vi "FluidtekPrensaCONidentLEDI_v17.vi"() -> ()   [LabVIEW 2026]
uses:
  <vilib>/DAQmx/write.llb/DAQmx Write (Analog DBL 1Chan 1Samp).vi
  <vilib>/DAQmx/read.llb/DAQmx Read (Analog 2D DBL NChan NSamp).vi
  <vilib>/DAQmx/read.llb/DAQmx Read (Digital 1D Bool NChan 1Samp 1Line).vi
  <vilib>/DAQmx/write.llb/DAQmx Write (Digital 1D Bool NChan 1Samp 1Line).vi
  <extravilib>/ChannelInstances/Stream-a[15](dbl)/Read With Abort.vi
  <extravilib>/ChannelInstances/Tag-a[28](dbl)/Read With Abort.vi
  <extravilib>/ChannelInstances/Tag-a[.](dbl)/Write With Abort.vi
  <extravilib>/ChannelInstances/Tag-a[.](dbl)/Read With Abort.vi
  <extravilib>/ChannelInstances/Stream-a[15](dbl)/Write With Abort.vi
  <extravilib>/ChannelInstances/Tag-a[28](dbl)/Write With Abort.vi
  <extravilib>/ChannelInstances/Stream-a[15](dbl)/EndpointRead.vi
  <extravilib>/ChannelInstances/Stream-a[15](dbl)/Endpoint.vi
  GlobalesPrensa.vi
  <vilib>/Utility/file.llb/Write Delimited Spreadsheet (DBL).vi
  <vilib>/DAQmx/create/channels.llb/DAQmx Create Channel (AO-Voltage-Basic).vi
  <vilib>/DAQmx/miscellaneous.llb/DAQmx Fill In Error Info.vi
  <vilib>/DAQmx/create/channels.llb/DAQmx Create Channel (AI-Voltage-Basic).vi
  <vilib>/DAQmx/configure/timing.llb/DAQmx Timing (Sample Clock).vi
  <vilib>/DAQmx/create/channels.llb/DAQmx Create Channel (DO-Digital Output).vi
  <vilib>/DAQmx/create/channels.llb/DAQmx Create Channel (DI-Digital Input).vi
  <extravilib>/ChannelInstances/Tag-a[.](dbl)/Instantiate.vi
  <extravilib>/ChannelInstances/Stream-a[15](dbl)/Instantiate.vi
  <extravilib>/ChannelInstances/Stream-a[15](dbl)/)Channel.vi
  <resource>/ChannelSupport/_ChannelSupport/WaitIfNeeded.vi
  <extravilib>/ChannelInstances/Tag-a[28](dbl)/Instantiate.vi
  <extravilib>/ChannelInstances/Tag-a[28](dbl)/EndpointRead.vi
  <extravilib>/ChannelInstances/Tag-a[.](dbl)/Endpoint.vi
  <extravilib>/ChannelInstances/Tag-a[.](dbl)/EndpointRead.vi
  <extravilib>/ChannelInstances/Tag-a[28](dbl)/Endpoint.vi
  <extravilib>/ChannelInstances/Tag-a[28](dbl).lvlib
  <extravilib>/ChannelInstances/Tag-a[.](dbl).lvlib
  <extravilib>/ChannelInstances/Stream-a[15](dbl).lvlib
  <vilib>/ptbypt/NI_PtbyPt.lvlib
panel:
  out "Archivo":path
  in  "PARO DE EMERGENCIA":bool
  out "time/iteration (ms)":u32=210
  in  "Tab Control 3":enum32{"ENSAYO", "REGISTRO"}(tab)
  in  "Tipo ensayos":u16(ring)=1 items=["Flexotraccion en losas", "Tenacidad Vigas"]
  in  "Rampa (mm/min)":dbl=0.1 min=0.0 max=30.0 format="%.3f"
  in  "Rampa (kN/min)":dbl=0.1 min=0.0 max=20.0 format="%.2f"
  in  "Limite fuerza (kN)":dbl=3.0 min=0.0 max=150.0 format="%.2f"
  in  "Limite posicion (mm)":dbl=145.0 min=0.0 max=150.0 format="%.2f"
  in  "Tiempo carga (s)":dbl=3.0 min=0.0 max=300.0 format="%.2g"
  out "Tiempo (s)":dbl format="%.2f"
  in  "Iniciar ensayo":bool
  out "Velocidad norma (mm/min)  2":string="0.05 - 0.1"
  in  "Tenacidad en vigas":u16(ring) items=["ASTM 1609 con100x100x350", "ASTM 1609 con150x150x500", "EFNARC 1996", "VIGAS 14651", "ENS. BARCELONA"]
  in  "Aplicar velocidad de norma":bool
  out "Estado del ensayo":dbl(ring) items=["REPOSO", "CARGA (rampa)", "MANTENIENDO CARGA", "DESCARGA", "RETORNO / FIN", "FALLA - ENSAYO DETENIDO", ""]
  in  "Flexotracción en losas":u16(ring)=3 items=["EFNARC 1996", "EFNARC 1999", "EFNARC 14488-5", "ASTM 1550"]
  out "Velocidad norma (mm/min)":dbl=4.0
  in  "IPAddress QuantumX":string="172.31.236.115"
  out "LicenseIsValid":bool
  in  "Registrar":bool
  in  "ID manual (0=auto)":i32
  in  "Tipo":string
  in  "INFLE":dbl
  in  "Detener registro":bool
  in  "Tab Control 2":T1(tab)
  out "Presión B (bar)":dbl=31.47939829954219 format="%.2f"
  out "Presión A (bar)":dbl=47.7049180327869 format="%.2f"
  out "Vertical Progress Bar":dbl(slide)=3.0
  in  "Tab Control":enum32{"Desplazamiento", "Fuerza"}(tab)
  out "control signals":dynamicdata(graph)=[{"t0"=timestamp(3594752785.1434503 s since 1904-01-01), "dt"=1.0, "Y"=[3.0]}, {"t0"=timestamp(3594752785.1434503 s since 1904-01-01), "dt"=1.0, "Y"=[3.0680651042487943]}]
  in  "Posicion deseada (mm)":dbl(slide)=3.0 min=2.0 max=150.0 scale format="%#_2f"
  in  "Fuerza deseada (kN)":dbl=0.5 min=0.0 max=150.0 format="%.2f"
  out "Fuerza actual (KN)":dbl format="%.2f"
  out "Posicion actual (mm)":dbl format="%.2f"
  in  "Tipo control":u16(ring) items=["Desplazamiento", "Fuerza"]
  out "fuerza desplazamiento":cluster{dbl[], dbl[]}(graph)
  out "Rigidez estimada (kN/mm)":dbl
  out "Carga maxima (kN)":dbl
  out "Progreso mantenimiento":dbl(slide) scale=0.0..100.0
  out "Tiempo restante carga (s)":dbl
  out "Falla":bool
  out "Causa de la falla":dbl(ring) items=["Sin falla", "CAIDA DE CARGA (rotura)", "SOBRECARGA", "LIMITE DE POSICION", "PARO DE EMERGENCIA", "LIMITE DEL SISTEMA (160 kN)", "BOMBA DETENIDA", "LIMITE POR PRESIONES (160 kN)"]
  out "Proteccion de fuerza activa":bool
  in  "Vel. aproximacion (mm/min)":dbl=50.0 min=0.1 max=50.0
  in  "Fmax fuera de ensayo (kN)":dbl=1.0 min=0.2 max=50.0
  out "UPH energizada":bool=TRUE
  out "Nivel tanque":bool
  out "Estado de  filtro":bool=TRUE
  out "Sobrecorriente":bool
  in  "Stop":bool
  out "Estado de motor":bool
  in  "Apagar":bool
  in  "Encender":bool
  in  "Sin proteccion de carga":bool
  out "Consigna posicion interna (mm)":dbl
  out "Parametros avanzados":dbl(ring) items=["POR DEFECTO (bloqueados)", "PERSONALIZADOS (activos)"]
  in  "Codigo acceso":dbl
  in  "Kf lazo fuerza (1/s)":dbl=0.5
  in  "Kx lazo posicion (V/mm)":dbl=30.0
  in  "Ti lazo posicion (s)":dbl=1.5
  # "PB"
  # "PA"
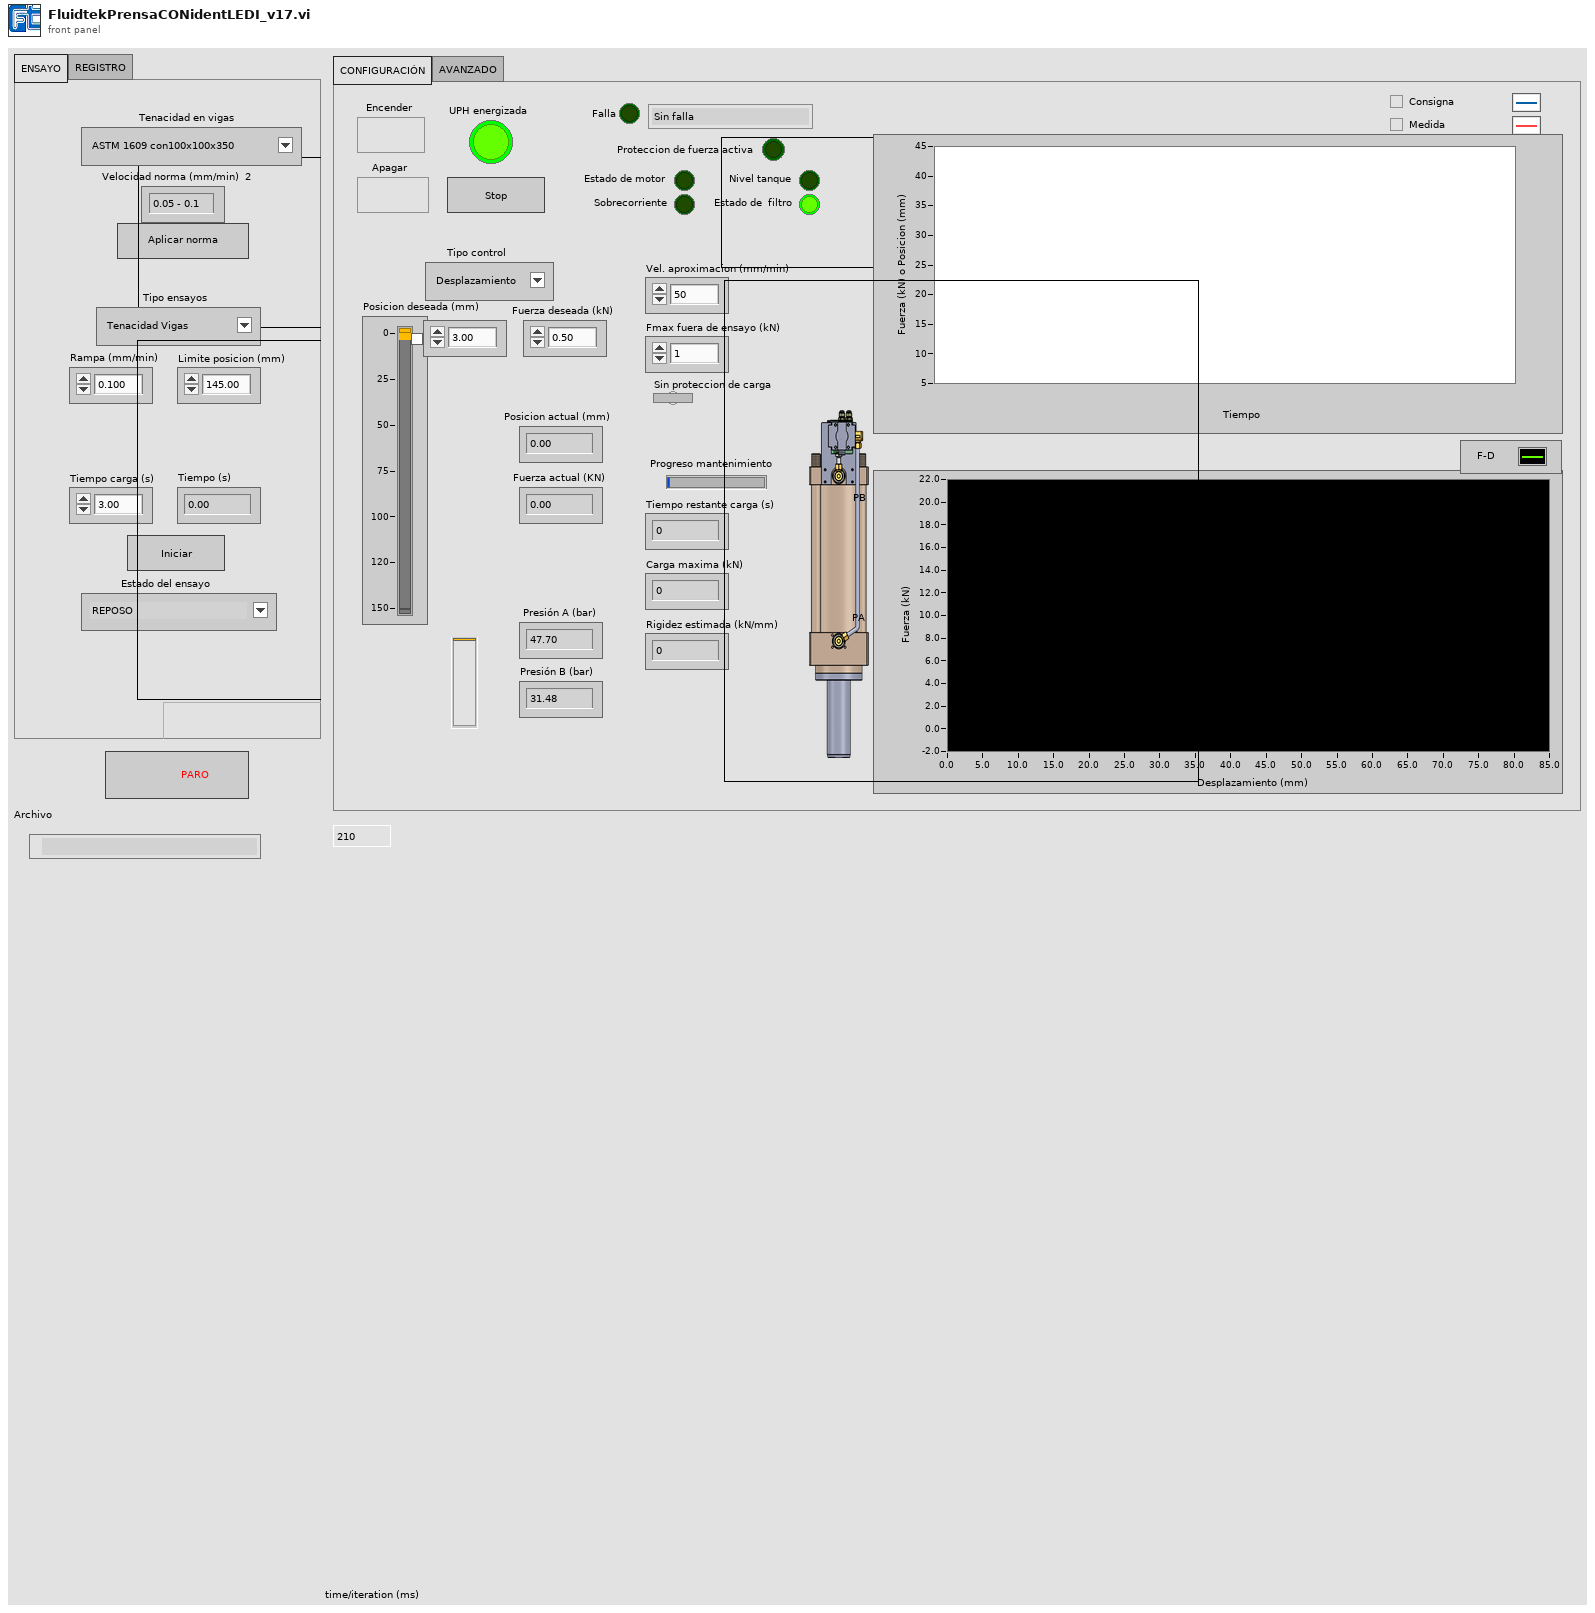
[diagram p1: front panel]
types:
  T1 = enum32{"CONFIGURACIÓN", "AVANZADO", "identificación (no modificar)"}
  T2 = cluster{"Devices":refnum<k24>[], "Signals":refnum<k24>[]}
  T3 = typedef "Tag-a[28](dbl).lvlib/))Channel.ctl" = refnum<queue>
  T4 = typedef "Stream-a[15](dbl).lvlib/)Channel.ctl" = refnum<queue>
  T5 = enum8{"Enabled", "Disabled", "Disabled and Grayed Out"}
  T6 = typedef "Tag-a[.](dbl).lvlib/))Channel.ctl" = refnum<queue>
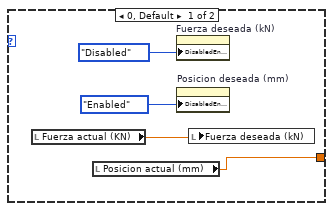
[diagram p9: hidden frame]
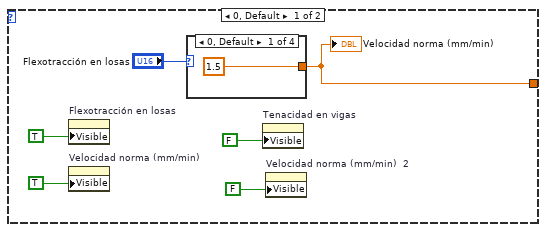
[diagram p10: hidden frame]
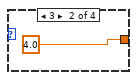
[diagram p11: hidden frame]
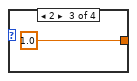
[diagram p12: hidden frame]
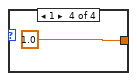
[diagram p13: hidden frame]
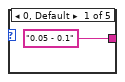
[diagram p14: hidden frame]
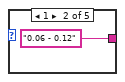
[diagram p15: hidden frame]
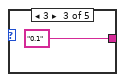
[diagram p16: hidden frame]
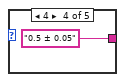
[diagram p17: hidden frame]
diagram:
  w93 = 0 items=["one channel for each line", "one channel for all lines"] ("line grouping")
  w100 = 0 items=["one channel for each line", "one channel for all lines"] ("line grouping")
  w103 = 10348 items=["Volts"=10348, "From Custom Scale"=10065] ("units")
  w106 = -1 items=["Default"=-1, "RSE"=10083, "NRSE"=10078, "Differential"=10106, "Pseudodifferential"=12529] ("input terminal configuration")
  w114 = 10348 items=["Volts"=10348, "From Custom Scale"=10065] ("units")
  w112 = 10106 items=["Default"=-1, "RSE"=10083, "NRSE"=10078, "Differential"=10106, "Pseudodifferential"=12529] ("input terminal configuration")
  w108 = 10123 items=["Finite Samples"=10178, "Continuous Samples"=10123, "Hardware Timed Single Point"=12522] ("sample mode")
  # "Convert device reference to array of device references\n(since ConnectDevice.vi expects an array of devices)..."
  # "Disconnect devices"
  # "Set samplerate and filter frequency for all selected signals."
  # "Initialize HBM Common API for LabVIEW"
  # "End API usage"
  # "Stop DAQ"
  # "Run data acquisition for 10 sec. DAQ-loop: Update signals and do anything with the  measurement values.\n(Here: show first signal in diagram)"
  # "Start DAQ"
  # "Prepare DAQ"
  # "v14: senales [0,1,2,3] -> lazo lee 1,2,3 = W100 (conector 2), Tempsonic (conector 3), Celda via Krenel (conector 4). Filtro 20 Hz, 50 Hz"
  # "Get all signals of the devices"
  # "Connect devices"
  # "Use certain QuantumX device"
  # "Assign the signals...."
  n1 = call <userlib>:"Init.vi"() -> ("LicenseIsValid"=→"LicenseIsValid":bool, "Error out"=w53:errorcluster)  [unwired: 8 in, 1 out]
  n2 = call <userlib>:"QuantumX_Device.vi"("Error in"=w53, "IPAddress"="IPAddress QuantumX") -> ("Error out"=w54:errorcluster, "Device"=w51:refnum<k24>)  [unwired: 6 in]
  n3 = Build Array(w51) -> (w50:refnum<k24>[])
  n4 = call <userlib>:"ConnectDevice.vi"("Error in"=w54, "Devices"=w50) -> ("Error out"=w76:errorcluster, "Devices"=w75:refnum<k24>[])  [unwired: 7 in, 1 out]
  n5 = call <userlib>:"GetSignals.vi"("Error in"=w76, "Devices"=w75) -> ("Error out"=w70:errorcluster, "DevicesAndSignals"=w71:T2)  [unwired: 8 in]
  n6 = Unbundle By Name(w71) -> ("Devices"=w64:refnum<k24>[], "Signals"=w68:refnum<k24>[])
  n7 = Index Array(array=w68, index #1=0 ("Index"), index #2=1 ("Index"), index #3=2 ("Index"), index #4=3 ("Index")) -> (element #1=w67:refnum<k24>, element #2=w66:refnum<k24>, element #3=w59:refnum<k24>, element #4=w58:refnum<k24>)
  n8 = Build Array(w67, w66, w59, w58) -> (w65:refnum<k24>[])
  n9 = Bundle(cluster=w71, "Devices"=w64, "Signals"=w65) -> (w72:T2)
  n10 = Unbundle By Name(w72) -> ("Signals"=w88:refnum<k24>[])
  n11 = case shown="No Error" w70 {
    tunnel: w70 -> [w122 w128]
    tunnel: w88 -> [w121 _]
    tunnel: [w120 w128] -> w87
    frame No Error {
      # "Filter frequency:"
      # "Samplerate:"
      n12 = for {
        tunnel: w122 -> [w127]
        tunnel: 50.0 ("SampleRate") -> [w126]
        tunnel: 20.0 ("FilterFrequency") -> [w125]
        tunnel: w121 -> [w124] mode=indexing
        tunnel: [w123] -> w120
        stop <- w123 stop-if-true
        n13 = call <userlib>:"ConfigSignal.vi"("Error in"=w127, "SampleRate"=w126, "FilterFrequency"=w125, "Signal"=w124) -> ("Error out"=w123:errorcluster)  [unwired: 7 in]
      }
    }
    frame Error {
    }
  }
  n14 = call <userlib>:"AssignSignals.vi"("Error in"=w87, "DevicesAndSignals"=w72) -> ("Error out"=w85:errorcluster, "DevicesAndSignals"=w86:T2)  [unwired: 8 in]
  n15 = call <userlib>:"PrepareDAQ.vi"("Error in"=w85, "DevicesAndSignals"=w86) -> ("Error out"=w82:errorcluster, "DaqMeasurement"=w83:refnum<k24>, "DevicesAndSignals"=w84:T2)  [unwired: 7 in]
  n16 = call <userlib>:"StartDaq.vi"("DevicesAndSignals"=w84, "DaqMeasurement"=w83, "AcquisitionMode"=2, "Error in"=w82) -> ("DevicesAndSignals"=w79:T2, "DaqMeasurement"=w80:refnum<k24>, "Error out"=w81:errorcluster)  [unwired: 7 in, 2 out]
  n17 = while {
    tunnel: w80 -> [w184]
    tunnel: w79 -> [w183]
    tunnel: [w179] -> w78
    tunnel: [w178] -> w77
    tunnel: w81 -> [w185]
    tunnel: [w177] -> w46
    shift-right: [w145] -> _
    shift-left: 0 -> [w170]
    shift-right: [w136] -> _
    shift-left: FALSE ("Registrar") -> [w141]
    shift-right: [w140] -> _
    shift-left: _ -> [w142]
    stop <- w131 stop-if-true
    n18 = global read "GlobalesPrensa.vi" "Salir"() -> (w130:bool)
    n19 = Get Date/Time In Seconds() -> (seconds since 1Jan1904=w153:timestamp)
    n20 = Format Into String(format string="D:\\\\%<%Y>T\\\\%03d-%<%Y>T", w153, "INFLE", w153) -> (resulting string=w155:string)  [unwired: 2 in, 1 out]
    n21 = Or(x=w130, y="Detener registro") -> (x .or. y?=w131:bool)
    n22 = String To Path(string=w155) -> (path=w158:path)
    n23 = Create Folder(path (use dialog)=w158) -> (error out=w156:errorcluster)  [unwired: 2 in, 2 out]
    n24 = Format Into String(format string="%s P*", "Tipo") -> (resulting string=w159:string)  [unwired: 2 in, 1 out]
    n25 = call <vilib>:"Clear Errors.vi"("error in (no error)"=w156) -> ("error out"=w157:errorcluster)  [unwired: 5 in, 1 out]
    n26 = List Folder(path=w158, pattern=w159, error in=w157) -> (path out=w168:path, filenames=w160:string[])  [unwired: 1 in, 2 out]
    n27 = Not(x=w141) -> (.not. x?=w147:bool)
    n28 = for {
      tunnel: w160 -> [w212] mode=indexing
      tunnel: [w210] -> w161 mode=indexing
      n29 = Scan From String(format string="%s P%d", input string=w212) -> (error out=w209:errorcluster, output 2=w210:i32)  [unwired: 5 in, 2 out]
      n30 = call <vilib>:"Clear Errors.vi"("error in (no error)"=w209) -> ()  [unwired: 5 in, 2 out]
    }
    n31 = Array Max & Min(array=w161) -> (max value=w162:i32)  [unwired: 3 out]
    n32 = Greater Than 0?(x="ID manual (0=auto)") -> (x > 0?=w164:bool)
    n33 = Increment(x=w162) -> (x+1=w163:i32)
    n34 = Select(t="ID manual (0=auto)", s=w164, f=w163) -> (s? t:f=w166:i32)
    n35 = global read "GlobalesPrensa.vi" "Ensayando"() -> (w137:bool)
    n36 = global read "GlobalesPrensa.vi" "InfoEnsayo"() -> (w134:string)
    n37 = Format Into String(format string="%s P%d.csv", "Tipo", w166) -> (resulting string=w167:string)  [unwired: 2 in, 1 out]
    n38 = Or(x="Registrar", y=w137) -> (x .or. y?=w136:bool)
    n39 = Build Path(base path=w168, name or relative path=w167) -> (appended path=w143:path)
    n40 = Get Date/Time In Seconds() -> (seconds since 1Jan1904=w135:timestamp)
    n41 = And(x=w136, y=w147) -> (x .and. y?=w148:bool)
    n42 = Select(t=w142, s=w141, f=w143) -> (s? t:f=w140:path)
    "Archivo" <- w140
    n43 = Format Into String(format string="Fecha\t%<%Y-%m-%d %H:%M:%S>T\nNorma\t%s\nFrecuencia (Hz)\t50\nRunning Time\tDeflection\tDisplacement\tLoad\ns\tmm\tmm\tkN\n", w135, w134) -> (resulting string=w133:string)  [unwired: 2 in, 1 out]
    n44 = case shown="True" w148 {
      tunnel: [_ w207] -> w149
      tunnel: w140 -> [_ w205]
      tunnel: w133 -> [_ w206]
      frame False {
      }
      frame True {
        (unwired) "" ("text")
        (unwired) errorcluster {"status"=FALSE, "code"=0, "source"=""} ("error in")
        (unwired) "" ("prompt (Choose or enter file path)")
        # "t (s)\\testado\\tconsigna\\tF (kN)\\tx (mm)\\txsp (mm)\\tu (V)\\tkh (kN/mm)\\tdt (s)\\tfalla\\tcausa\\tprot\\n"
        n45 = Path To String(path=w205) -> (string=w204:string)
        n46 = Search and Replace String(replace all?=FALSE ("replace all? (F)"), case sensitive?=FALSE ("ignore case? (F)"), input string=w204, search string=".csv", replace string="_control.csv" ("replace string (\"\")"), offset=0 ("offset (0)"), error in=errorcluster {"status"=FALSE, "code"=0, "source"=""} ("error in (no error)")) -> (result string=w197:string)  [unwired: 1 in, 3 out]
        n47 = String To Path(string=w197) -> (path=w196:path)
        n48 = Write to Text File(file (use dialog)=w196, text="t (s)\testado\tconsigna\tF (kN)\tx (mm)\txsp (mm)\tu (V)\tkh (kN/mm)\tdt (s)\tfalla\tcausa\tprot\tpA (bar)\tpB (bar)\tFp (kN)\n") -> (error out=w194:errorcluster)  [unwired: 2 in, 2 out]
        n49 = flat-sequence {
          tunnel: w196 -> [w208]
          tunnel: w194 -> [_]
          frame #0 {
            n50 = global write "GlobalesPrensa.vi" "ArchivoControl"(w208) -> ()
          }
        }
        n51 = Write to Text File(file (use dialog)=w205, text=w206) -> (error out=w207:errorcluster)  [unwired: 2 in, 2 out]
      }
    }
    n52 = call <userlib>:"UpdateMeasurementValues.vi"("Error in"=w185, "DaqMeasurement"=w184, "DevicesAndSignals"=w183) -> ("Error out"=w180:errorcluster, "DaqMeasurement"=w181:refnum<k24>, "DevicesAndSignals"=w182:T2)  [unwired: 6 in]
    n53 = for {
      N: 3 -> [_]
      shift-right: [w224] -> w178
      shift-left: w182 -> [w228]
      shift-right: [w225] -> w179
      shift-left: w181 -> [w227]
      shift-right: [w223] -> w177
      shift-left: w180 -> [w226]
      tunnel: [w218] -> w129 mode=indexing
      i -> [w221]
      n54 = Add(x=w221, y=1.0) -> (x+y=w220:dbl)
      n55 = call <userlib>:"GetMeasurementValues.vi"("Error in"=w226, "Index"=w220, "DaqMeasurement"=w227, "DevicesAndSignals"=w228) -> ("Error out"=w223:errorcluster, "Waveform"=w219:waveform(dbl), "DaqMeasurement"=w225:refnum<k24>, "DevicesAndSignals"=w224:T2)  [unwired: 2 in, 2 out]
      n56 = Unbundle By Name(w219) -> ("Y"=w218:dbl[])
    }
    n57 = Array Size(array=w129) -> (size(s)=w173:i32[])
    n58 = Index Array(array=w173, index=1) -> (element=w171:i32)
    n59 = for {
      N: w171 -> [_]
      tunnel: [w215] -> w169 mode=indexing
      tunnel: w170 -> [w213]
      i -> [w217]
      n60 = Add(x=w217, y=w213) -> (x+y=w216:i32)
      n61 = Multiply(x=w216, y=0.02) -> (x*y=w215:dbl)
    }
    n62 = Add(x=w170, y=w171) -> (x+y=w146:i32)
    n63 = Select(t=w146, s=w136, f=0) -> (s? t:f=w145:i32)
    n64 = case shown="True" w136 {
      tunnel: w129 -> [_ w193]
      tunnel: w169 -> [_ w192]
      tunnel: w149 -> [_ w187]
      tunnel: w140 -> [_ w186]
      frame False {
      }
      frame True {
        n65 = Insert Into Array(array=w193, index (row)=0, new element=w192) -> (w190:dbl[][])  [unwired: 1 in]
        n66 = call-poly <vilib>:"Write Delimited Spreadsheet.vi"("file path (dialog if empty)"=w186, "2D data"=w190, "append to file? (new file:F)"=TRUE, "error in (no error)"=w187, "transpose? (no:F)"=TRUE) -> ()  [unwired: 9 in, 2 out]
      }
    }
    n67 = Wait Until Next ms Multiple(millisecond multiple=u32 20 ("Vielfache von ms")) -> ()  [unwired: 1 out]
  }
  n68 = while {
    tunnel: [w230] -> w44
    tunnel: [w230] -> w43
    tunnel: [w230] -> w42
    i -> [w235]
    stop <- w233 continue-if-true
    n69 = call <vilib>:"DAQmx Reserve Network Device.vi"("device in"=tag "cDAQ9184-1ADC24C", "override reservation?"=TRUE, "error in"=errorcluster {"status"=FALSE, "code"=0, "source"=""}) -> ("error out"=w230:errorcluster)  [unwired: 11 in, 1 out]
    n70 = Unbundle By Name(w230) -> ("status"=w232:bool)
    n71 = Less?(x=w235, y=30) -> (x < y?=w234:bool)
    n72 = Wait (ms)(milliseconds to wait=u32 2000) -> ()  [unwired: 1 out]
    n73 = And(x=w232, y=w234) -> (x .and. y?=w233:bool)
  }
  n74 = call-poly <vilib>:"DAQmx Create Virtual Channel.vi"("maximum value"=10.0, "minimum value"=0.0, "input terminal configuration"=w112, "physical channels"=tag "PrensaLEDI_AI/ai0:3", "units"=w114, "error in"=w42) -> ("task out"=w115:refnum<k21>, "error out"=w116:errorcluster)  [unwired: 8 in]
  n75 = call-poly <vilib>:"DAQmx Create Virtual Channel.vi"("maximum value"=10.0, "minimum value"=-10.0, "output terminal configuration"=w106, "physical channels"=tag "PrensaLEDI_AO/ao0", "units"=w103, "error in"=w42) -> ("task out"=w107:refnum<k21>, "error out"=w105:errorcluster)  [unwired: 8 in]
  n76 = call-poly <vilib>:"DAQmx Create Virtual Channel.vi"("lines"=tag "PrensaLEDI_DI/port0/line0:7", "line grouping"=w100, "error in"=w44) -> ("task out"=w97:refnum<k21>, "error out"=w98:errorcluster)  [unwired: 11 in]
  n77 = call-poly <vilib>:"DAQmx Create Virtual Channel.vi"("lines"=tag "PrensaLEDI_DO/port0/line0:7", "line grouping"=w93, "error in"=w43) -> ("task out"=w94:refnum<k21>, "error out"=w95:errorcluster)  [unwired: 11 in]
  n78 = call <vilib>:"DAQmx Start Task.vi"("task/channels in"=w107, "error in"=w105) -> ("task out"=w40:refnum<k21>, "error out"=w41:errorcluster)  [unwired: 12 in]
  n79 = call <vilib>:"Clear Errors.vi"("error in (no error)"=w46) -> ("error out"=w45:errorcluster)  [unwired: 5 in, 1 out]
  n80 = call <vilib>:"DAQmx Start Task.vi"("task/channels in"=w97, "error in"=w98) -> ("task out"=w25:refnum<k21>, "error out"=w17:errorcluster)  [unwired: 12 in]
  n81 = call <vilib>:"DAQmx Start Task.vi"("task/channels in"=w94, "error in"=w95) -> ("task out"=w37:refnum<k21>, "error out"=w18:errorcluster)  [unwired: 12 in]
  n82 = call-poly <vilib>:"DAQmx Timing.vi"("task/channels in"=w115, "sample mode"=w108, "samples per channel"=500000, "rate"=200000.0, "error in"=w116) -> ("task out"=w92:refnum<k21>, "error out"=w91:errorcluster)  [unwired: 9 in]
  n83 = call <userlib>:"StopDaq.vi"("Error in"=w45, "DaqMeasurement"=w78, "DevicesAndSignals"=w77) -> ("Error out"=w57:errorcluster, "DevicesAndSignals"=w56:T2)  [unwired: 7 in]
  n84 = call-poly <vilib>:"DAQmx Write.vi"("task/channels in"=w40, "data"=-0.5, "error in"=w41) -> ("task out"=w36:refnum<k21>, "error out"=w15:errorcluster)  [unwired: 10 in, 1 out]
  n85 = call <vilib>:"DAQmx Start Task.vi"("task/channels in"=w92, "error in"=w91) -> ("task out"=w38:refnum<k21>, "error out"=w16:errorcluster)  [unwired: 12 in]
  n86 = call <userlib>:"DisconnectDevice.vi"("Error in"=w57, "DevicesAndSignals"=w56) -> ("Error out"=w55:errorcluster)  [unwired: 9 in]
  n87 = call <vilib>:"Simple Error Handler.vi"("error in (no error)"=w55) -> ("error out"=w74:errorcluster)  [unwired: 4 in, 4 out]
  n88 = Merge Errors(w18, w17, w16, w15) -> (w19:errorcluster)
  n89 = call <userlib>:"DisposeApi.vi"("Error in"=w74) -> ()  [unwired: 10 in, 1 out]
  n90 = global write "GlobalesPrensa.vi" "Salir"(FALSE ("Salir")) -> ()
  n91 = while {
    tunnel: w38 -> [w280]
    tunnel: w37 -> [w270]
    tunnel: w36 -> [w268]
    tunnel: dbl[] [0.0, 0.0, 0.0, 0.0, 0.0, 0.0, 0.0, 0.0, 0.0, 0.0, 0.0, 0.0, 0.0, 0.0, 0.0, 0.0, 0.0] -> [w265]
    tunnel: dbl[] [0.0, 0.0, 0.0, 0.0, 0.0, 0.0, 0.0, 0.0] -> [w264]
    tunnel: [w263] -> w32
    tunnel: [w262] -> w31
    tunnel: w25 -> [w260]
    tunnel: [w259] -> w22
    tunnel: [w258] -> w21
    tunnel: [w257] -> w20
    tunnel: w19 -> [w256]
    tunnel: [w243] -> w13
    tunnel: [w242] -> w2
    tunnel: w1 -> [w241]
    stop <- w244 stop-if-true
    n92 = call <extravilib>:"Read.vi"("channel"=w241) -> ("element"=w240:dbl[])  [unwired: 1 in, 1 out]
    n93 = call-poly <vilib>:"DAQmx Read.vi"("task/channels in"=w280, "number of samples per channel"=4000, "error in"=w256) -> ("task out"=w258:refnum<k21>, "data"=w279:dbl[][], "error out"=w255:errorcluster)  [unwired: 10 in]
    n94 = call-poly <vilib>:"DAQmx Read.vi"("task/channels in"=w260, "error in"=w255) -> ("task out"=w259:refnum<k21>, "data"=w261:bool[], "error out"=w254:errorcluster)  [unwired: 11 in]
    n95 = Boolean To (0,1)(Boolean=w261) -> (0, 1=w281:i16[])
    n96 = To Double Precision Float(number=w281) -> (double precision float=w278:dbl[])
    n97 = formula code="/* ===========================================================================\n   NODO ENTRADAS - prensa Fluidtek, VI v17\n   Primer Formula Node del lazo de maquina: promedia, escala y valida las cuatro\n   lecturas analogicas de cada paso.\n   ===========================================================================\n\n   TERMINALES\n     Entrada   V   voltios, arreglo 2D [canal][muestra] de DAQmx Read\n                   \"Analog 2D DBL NChan NSamp\" sobre PrensaLEDI_AI/ai0:3\n                   (4 canales x 4000 muestras a 200 kS/s = 20 ms)\n     Salida    M   medidas (7), para el nodo PID\n\n   M[]  0 x   posicion del vastago [mm]            ai0, Temposonic   15 mm/V\n        1 F   fuerza de la celda [kN]               ai1               20 kN/V\n        2 pa  presion camara A, SIN vastago [bar]   ai2, TR44.2  (V - 1.9826)*12.5\n        3 pb  presion camara B, CON vastago [bar]   ai3, TR49.2  (V - 1.9682)*50\n        4 ok  1 = posicion y fuerza validas. Con 0 el PID manda u_seguro y, si\n              hay ensayo, lo deja en FALLA\n        5 aviso de presiones (no detiene nada mientras el corte por presiones\n              este desactivado): 0 ninguno, 1 camara A, 2 camara B, 3 las dos\n        6 dt  periodo del paso [s] = muestras leidas / fs\n\n   El promedio de 20 ms es el filtro de las medidas: anula 50 Hz y sus armonicos\n   y deja el ruido de posicion muy por debajo de 0.1 mm.\n   =========================================================================== */\n\nint32 i, n;\nfloat64 fs, v0, v1, v2, v3, v_min, v_max, v_lazo;\nfloat64 M[7];\n\nfs     = 200000;    /* muestras/s por canal: la misma del DAQmx Timing del diagrama */\nv_min  = -0.5;      /* V: por debajo, posicion o fuerza no son creibles */\nv_max  = 10.5;      /* V: por encima, entrada saturada o desconectada */\nv_lazo = 1.5;       /* V: un transductor 4-20 mA sano da >= 2 V; menos = lazo abierto o sin alimentar */\n\n/* promedio de cada canal */\nn = 0;\nif (sizeOfDim(V,0)>=4) n = sizeOfDim(V,1);\nv0=0; v1=0; v2=0; v3=0;\nfor (i=0; i<n; i++) {\n    v0 = v0 + V[0][i];\n    v1 = v1 + V[1][i];\n    v2 = v2 + V[2][i];\n    v3 = v3 + V[3][i];\n}\nif (n>0) { v0=v0/n; v1=v1/n; v2=v2/n; v3=v3/n; }\n\n/* escalas */\nM[0] = 15*v0;\nM[1] = 20*v1;\nM[2] = (v2-1.9826)*12.5;\nM[3] = (v3-1.9682)*50;\n\n/* validez de posicion y fuerza: hay muestras, no son NaN y estan en rango */\nM[4] = 1;\nif (n<1) M[4] = 0;\nif (!(v0==v0) || !(v1==v1)) M[4] = 0;\nif (v0<v_min || v0>v_max || v1<v_min || v1>v_max) M[4] = 0;\n\n/* aviso de presiones: lazo abierto, saturado o NaN */\nM[5] = 0;\nif (!(v2==v2) || v2<v_lazo || v2>v_max) M[5] = M[5] + 1;\nif (!(v3==v3) || v3<v_lazo || v3>v_max) M[5] = M[5] + 2;\n\n/* periodo del paso: lo fija el reloj de muestreo, no el del PC */\nM[6] = n/fs;"("V"=w279) -> ("M"=w276:dbl[])
    n98 = feedback #1(w264) -> (w277:dbl[])
    n99 = formula code="/* ===========================================================================\n   NODO UPH - prensa Fluidtek, VI v17\n   Segundo Formula Node del lazo de maquina: unidad hidraulica y seguridad.\n   Lee las entradas digitales, decide la orden de la bomba y arma las salidas\n   digitales.\n   ===========================================================================\n\n   TERMINALES\n     Entradas  D   las 8 entradas digitales como 0/1 (PrensaLEDI_DI/port0/line0:7)\n               C   comandos del panel (los mismos del nodo PID)\n               Gp  la salida G del paso anterior (vacia en la primera iteracion)\n     Salidas   O   las 8 salidas digitales como 0/1 (PrensaLEDI_DO/port0/line0:7)\n               G   UPH y seguridad (8), para el nodo PID y para Gp\n\n   D[]  0 seta de emergencia (1 = segura)   1 nivel de aceite (1 = OK)\n        2 filtro en linea (1 = limpio)      5 guardamotor GM1 (1 = disparado o apagado)\n        7 confirmacion de marcha, KM1 (1 = bomba en marcha)\n   C[]  2 PARO del panel   3 encender (pulso)   4 apagar (pulso)   5 salir (Stop)\n   O[]  0 orden de bomba (K1 -> KM1)\n        2 \"salida contactor2\" (K3): 1 con la seta pulsada o al salir, como en la v16\n        5 alimentacion de los transductores de presion (K6): siempre 1\n   G[]  0 seta (1 = segura)   1 bomba en marcha (DI7)   2 orden de bomba\n        3 nivel   4 filtro   5 guardamotor   6 salir\n        7 pasos seguidos con orden de bomba y sin confirmacion de marcha\n\n   ORDEN DE BOMBA  Enclavamiento con PRIORIDAD AL APAGADO: seta pulsada, PARO,\n   Apagar o Salir la ponen a 0 aunque llegue Encender en el mismo paso; Encender\n   la pone a 1; si no hay orden, conserva la anterior. Sin entradas digitales o\n   sin comandos, la bomba queda apagada.\n\n   BOMBA QUE NO CONFIRMA  Si hay orden y DI7 no confirma la marcha durante 2 s\n   (guardamotor disparado, contactor que no entra), la orden se retira: asi la\n   bomba no arranca sola al rearmar el guardamotor. Hay que pulsar Encender.\n   =========================================================================== */\n\nint32 i;\nfloat64 seta, nivel, filtro, guarda, marcha;\nfloat64 paro, encender, apagar, salir, bomba, sin_marcha, pasos_conf;\nfloat64 O[8], G[8];\n\npasos_conf = 100;   /* pasos de 20 ms sin confirmacion de marcha antes de retirar la orden (2 s) */\n\n/* entradas digitales: sin lectura, seta pulsada y todo en falta */\nseta=0; nivel=0; filtro=0; guarda=1; marcha=0;\nif (sizeOfDim(D,0)>=8) {\n    seta=D[0]; nivel=D[1]; filtro=D[2]; guarda=D[5]; marcha=D[7];\n}\n\n/* comandos: sin panel, como si se pidiera PARO */\nparo=1; encender=0; apagar=0; salir=0;\nif (sizeOfDim(C,0)>=20) {\n    paro=C[2]; encender=C[3]; apagar=C[4]; salir=C[5];\n}\n\n/* orden de bomba: la anterior, salvo orden nueva; el apagado manda */\nbomba = 0; sin_marcha = 0;\nif (sizeOfDim(Gp,0)>=8) { bomba = Gp[2]; sin_marcha = Gp[7]; }\nif (encender>0.5) bomba = 1;\nif (seta<0.5 || paro>0.5 || apagar>0.5 || salir>0.5) bomba = 0;\n\n/* bomba que no confirma: con orden y sin marcha se cuenta; pasado el plazo se retira la orden */\nif (bomba>0.5 && marcha<0.5) sin_marcha = sin_marcha + 1;\nelse sin_marcha = 0;\nif (sin_marcha>pasos_conf) { bomba = 0; sin_marcha = 0; }\n\n/* salidas digitales */\nfor (i=0; i<8; i++) O[i] = 0;\nO[0] = bomba;\nif (seta<0.5 || salir>0.5) O[2] = 1;\nO[5] = 1;\n\n/* estado para el PID y para el paso siguiente */\nG[0]=seta;  G[1]=marcha;  G[2]=bomba;  G[3]=nivel;  G[4]=filtro;  G[5]=guarda;  G[6]=salir;\nG[7]=sin_marcha;"("D"=w278, "C"=w240, "Gp"=w277) -> ("O"=w272:dbl[], "G"=w267:dbl[])
    n100 = feedback-in #1(w267) -> ()
    n101 = Not Equal To 0?(x=w272) -> (x != 0?=w271:bool[])
    n102 = Index Array(array=w267, index=6) -> (element=w247:dbl)
    n103 = call-poly <vilib>:"DAQmx Write.vi"("task/channels in"=w270, "data"=w271, "error in"=w254) -> ("task out"=w262:refnum<k21>, "error out"=w253:errorcluster)  [unwired: 10 in, 1 out]
    n104 = call <vilib>:"High Resolution Relative Seconds.vi"() -> ("relative seconds"=w273:dbl)
    n105 = Greater?(x=w247, y=0.5) -> (0:w246:bool)
    n106 = feedback #2(w265) -> (w274:dbl[])
    n107 = formula code="/* ===========================================================================\n   NODO PID - prensa Fluidtek, VI v17 - cascada fuerza -> posicion\n   Tercer Formula Node del lazo de maquina (un paso cada 20 ms):\n       ENTRADAS (Entradas.c) -> M      UPH (Uph.c) -> G      panel -> C\n   ===========================================================================\n\n   QUE HACE\n     1. Genera la consigna sp segun el estado st (maquina de estados).\n     2. Lazo externo: convierte sp (posicion o fuerza) en consigna de posicion\n        x_ref. En fuerza se divide por la rigidez estimada rig [kN/mm].\n     3. Lazo interno: PI de posicion -> comando u [V] a la servovalvula.\n     4. Protecciones: celda (F_corte), sobrecarga, caida de carga, limite de\n        posicion, paro de emergencia (boton o seta), bomba detenida, presiones\n        (desactivado), medidas invalidas y comandos incompletos.\n\n   COMANDO SEGURO u_seguro = -0.5 V\n     0 V NO es reposo: el null de la servovalvula esta en -0.37 V, y a 0 V el\n     vastago se EXTIENDE ~8 mm/min mientras quede presion. Por eso el PARO, la\n     bomba detenida, la medida invalida y los limites de fuerza/presion no usan\n     0 V sino u_seguro, que queda por debajo del null aunque derive y retrae a\n     ~3 mm/min.\n\n   ESTADOS  st      0 reposo/aproximacion   1 carga   2 mantener   3 descarga\n                    4 retorno/fin           5 FALLA\n   CAUSAS   causa   0 ninguna  1 caida de carga  2 sobrecarga  3 limite de posicion\n                    4 paro de emergencia (boton PARO o seta)\n                    5 limite de la celda (F_corte)\n                    6 bomba detenida: FALLA en ensayo, aviso en reposo\n                    7 limite por presiones (pa >= pa_max o F_pres >= F_corte)\n   MODOS    modo    0 control de desplazamiento [mm]    1 control de fuerza [kN]\n\n   TERMINALES\n     Entradas  M   medidas, de ENTRADAS (7)   G   UPH y seguridad, de UPH (8)\n               C   comandos del panel (21)    S   estado del paso anterior (17)\n               tr  reloj de alta resolucion del PC [s] (solo para medir atrasos)\n     Salidas   u   comando de la servovalvula [V]\n               So  estado para el paso siguiente (17)\n               E   estado para la interfaz y el registro (28)\n\n   M[]  0 x [mm]   1 F [kN]   2 pa [bar] (camara A, SIN vastago)   3 pb [bar] (camara B,\n        CON vastago)   4 ok (1 = x y F validas)   5 aviso de presiones   6 dt [s]\n   G[]  0 seta (1 = segura)   1 bomba en marcha (DI7)   2 orden de bomba   3 nivel\n        4 filtro   5 guardamotor   6 salir   7 pasos con orden y sin marcha\n   C[]  0 modo   1 iniciar   2 PARO   3 encender   4 apagar   5 salir   6 sin proteccion\n        7 posicion deseada [mm]    8 fuerza deseada [kN]\n        9 limite de posicion [mm]  10 limite de fuerza [kN]\n        11 rampa [mm/min]          12 rampa [kN/min]         13 tiempo de carga [s]\n        14 velocidad de aproximacion [mm/min]   15 Fmax fuera de ensayo [kN]\n        16 codigo de acceso   17 Kx [V/mm]   18 Tix [s]   19 Kf [1/s]   20 latido\n   S[] -> So[]   (llega vacio o con ceros en la primera iteracion)\n        0 x_ref  1 rig   2 F_pico   3 integ   4 sp_prev   5 tr_prev\n        6 F_ref  7 x_ref_rig  8 x_inicio  9 u_prev  10 modo_prev  11 causa_act\n        12 st    13 f0   14 ts   15 ini_prev   16 t\n   E[]  0 t  1 st  2 sp  3 F  4 x  5 x_ref  6 u  7 rig  8 dt  9 falla  10 causa\n        11 prot  12 pa  13 pb  14 F_pres        (0-14: las columnas del CSV de control)\n        15 seta  16 bomba en marcha  17 orden de bomba  18 nivel  19 filtro\n        20 guardamotor  21 carga maxima [kN]  22 progreso [%]  23 tiempo restante [s]\n        24 parametros personalizados  25 aviso de presiones  26 dt del reloj del PC [s]\n        27 modo\n\n   PARAMETROS DEL PI   Por defecto Kx = 30 V/mm, Tix = 1.5 s, Kf = 0.5 1/s. Con el\n     codigo de acceso (C[16] = 2026) se usan los del panel, limitados a\n     Kx 1...100, Tix 0.1...60, Kf 0.05...5.\n\n   PARO (boton o seta) y BOMBA DETENIDA: salida u_seguro y controlador en\n   seguimiento (x_ref = x) con el integrador congelado, para que al soltar el\n   paro o al arrancar la bomba no haya salto. Al INICIAR un ensayo tampoco se\n   toca el integrador: el comando sigue en el null aprendido.\n\n   BASE DE TIEMPO: dt = M[6] (muestras leidas / 200 kS/s = 20 ms exactos) y t se\n   acumula aqui. El reloj del PC (tr) solo sirve para ver atrasos del lazo (E[26]).\n\n   El cuerpo (secciones 3 a 10) es el de PID.c v18 salvo el integrador, que ya no\n   se pone a cero al iniciar, al cambiar de modo ni en el PARO. Con ese unico\n   cambio aplicado a PID.c v18, y con seta = 1 y bomba en marcha, los dos dan\n   exactamente lo mismo (pruebas/arnes_v17.js).\n   =========================================================================== */\n\n\n/* ---------------------------------------------------------------------------\n   0. DECLARACIONES Y CONSTANTES\n   (el Formula Node no tiene #define: las constantes son variables)\n   --------------------------------------------------------------------------- */\n\n/* medidas (M), seguridad (G) y comandos (C) */\nfloat64 x, F, pa, pb, ok, aviso;\nfloat64 seta, uph;\nfloat64 modo, ini, paro, sinprot, spm, lim, rate, tc, xlim, vjog, Flib;\n/* parametros del PI y ajustes */\nfloat64 Kx, Tix, Kf, act, rig_ini, frac_caida, frac_sobre, v_retorno, du_max, par_ok;\n/* estado persistente (S) */\nfloat64 x_ref, rig, F_pico, integ, sp_prev, t_prev, F_ref, x_ref_rig, x_inicio;\nfloat64 u_prev, modo_prev, causa_act;\nfloat64 stp, f0p, tsp, inip, t;\n/* resultado del paso */\nfloat64 st, f0, ts, sp, prot, prog, trest, falla, causa;\n/* variables de trabajo */\nfloat64 med, dt, dt_real, v_aprox, F_lib, en_paro;\nfloat64 dif, vel_sp, dF_min, rig_nueva;\nfloat64 x_ref_ini, err;\nfloat64 F_pres, lim_pres;\n/* arreglos de salida */\nfloat64 So[17];\nfloat64 E[28];\n/* constantes de seguridad y de ajuste */\nfloat64 F_corte, pa_max, prot_pres_on, v_des, u_max, u_seguro, x_win, v_lenta;\nfloat64 rig_min, rig_max, alfa_rig, frac_freno, frac_pico_min, margen_xlim;\nfloat64 dF_min_rig, dx_min_rig, dx_sin_contacto;\nfloat64 cFpA, cFpB;\n/* codigos de estado y de causa */\nfloat64 ST_REPOSO, ST_CARGA, ST_MANTIENE, ST_DESCARGA, ST_RETORNO, ST_FALLA;\nfloat64 CAU_NINGUNA, CAU_CAIDA, CAU_SOBRECARGA, CAU_LIM_POS, CAU_PARO, CAU_FCORTE, CAU_BOMBA, CAU_PRESION;\n\nF_corte  = 160;     /* kN: corte por la celda. 160 kN ~ 80 bar con el cilindro 160/80: BAJAR (CLAUDE.md 6) */\npa_max   = 95;      /* bar: corte por presion de la camara A (el TR44.2 satura a 100 bar) */\nprot_pres_on = 0;   /* 0 = corte por presiones DESACTIVADO (desde 2026-11-03); 1 = activo */\nv_des    = 40;      /* kN/min: carga/descarga en fuerza fuera de ensayo y descarga en ensayo */\nu_max    = 10;      /* V: saturacion del comando (tambien umbral del anti-windup) */\nu_seguro = -0.5;    /* V: comando seguro (retrae ~3 mm/min). 0 V extiende: el null esta en -0.37 V */\nx_win    = 2;       /* mm: x_ref no se separa de x mas que esto */\nv_lenta  = 2;       /* mm/min: avance lento fuera de ensayo con compresion */\nrig_min  = 0.02;    /* kN/mm: rigidez estimada minima */\nrig_max  = 50;      /* kN/mm: rigidez estimada maxima */\nalfa_rig = 0.3;     /* filtro de la rigidez estimada */\nfrac_freno    = 0.25;   /* avance lento si F > frac_freno*F_lib (fuera de ensayo) */\nfrac_pico_min = 0.2;    /* la caida de carga solo cuenta si el pico fue > 20 % de lim */\nmargen_xlim   = 0.5;    /* mm: tolerancia sobre el limite de posicion xlim */\ndF_min_rig      = 0.05; /* kN: cambio minimo de fuerza para actualizar la rigidez */\ndx_min_rig      = 0.002;/* mm: cambio minimo de posicion para actualizar la rigidez */\ndx_sin_contacto = 5;    /* mm: mas que esto sin cambio de F = sin contacto */\nrig_ini      = 1;       /* kN/mm: rigidez inicial estimada */\nfrac_caida   = 0.3;     /* caida de carga que dispara FALLA (fraccion del pico) */\nfrac_sobre   = 1.2;     /* sobrecarga que dispara FALLA (fraccion de lim) */\nv_retorno    = 50;      /* mm/min: velocidad de retorno, todos los casos y modos */\ndu_max       = 40;      /* V/s: variacion maxima de la salida u */\n\n/* Fp = A_A*pa - A_B*pb con el cilindro 160/80 mm (kN/bar = A[m2]*100):\n   A_A = 201.06 cm2 (camara A, sin vastago), A_B = 150.80 cm2 (camara B, con vastago) */\ncFpA = 2.0106;\ncFpB = 1.5080;\n\nST_REPOSO = 0;  ST_CARGA = 1;  ST_MANTIENE = 2;  ST_DESCARGA = 3;  ST_RETORNO = 4;  ST_FALLA = 5;\nCAU_NINGUNA = 0;  CAU_CAIDA = 1;  CAU_SOBRECARGA = 2;  CAU_LIM_POS = 3;\nCAU_PARO = 4;  CAU_FCORTE = 5;  CAU_BOMBA = 6;  CAU_PRESION = 7;\n\n/* ---------------------------------------------------------------------------\n   0b. ENTRADAS: de los arreglos a variables con nombre\n   Si falta algun arreglo los valores son inertes y la seccion 12 deja el paso\n   en FALLA con u = u_seguro.\n   --------------------------------------------------------------------------- */\n\n/* medidas */\nx=0; F=0; pa=0; pb=0; ok=0; aviso=0; dt=0;\nif (sizeOfDim(M,0)>=7) {\n    x=M[0]; F=M[1]; pa=M[2]; pb=M[3]; ok=M[4]; aviso=M[5]; dt=M[6];\n}\nif (dt<=0 || dt>1) dt = 0.02;   /* sin medidas validas: periodo nominal */\n\n/* seguridad: sin datos de la UPH, seta pulsada y bomba detenida */\nseta=0; uph=0;\nif (sizeOfDim(G,0)>=7) { seta=G[0]; uph=G[1]; }\n\n/* comandos del panel. La consigna manual, la consigna final y la rampa dependen\n   del tipo de control */\npar_ok = sizeOfDim(C,0)>=20;\nmodo=0; ini=0; paro=1; sinprot=0; spm=0; lim=0; rate=0; tc=0; xlim=0; vjog=0; Flib=0;\nKx=0; Tix=1; Kf=0; act=0;\nif (par_ok) {\n    modo=C[0]; ini=C[1]; paro=C[2]; sinprot=C[6];\n    if (modo>0.5) { spm=C[8]; lim=C[10]; rate=C[12]; }\n    else          { spm=C[7]; lim=C[9];  rate=C[11]; }\n    xlim=C[9]; tc=C[13]; vjog=C[14]; Flib=C[15];\n    /* parametros del PI: por defecto, o los del panel con el codigo de acceso */\n    Kx=30; Tix=1.5; Kf=0.5;\n    if (C[16]==2026) {\n        Kx  = max(1,min(100,C[17]));\n        Tix = max(0.1,min(60,C[18]));\n        Kf  = max(0.05,min(5,C[19]));\n        act = 1;\n    }\n}\n\n/* ---------------------------------------------------------------------------\n   1. MEDICION ACTUAL Y ESTADO PERSISTENTE\n   --------------------------------------------------------------------------- */\n\n/* medicion del modo activo: posicion [mm] o fuerza [kN] */\nmed = x;\nif (modo>0.5) med = F;\n\n/* el estado llega vacio o con ceros en la primera iteracion: rig>0 indica estado valido */\nif (sizeOfDim(S,0)>=17 && S[1]>0) {\n    x_ref=S[0]; rig=S[1]; F_pico=S[2]; integ=S[3]; sp_prev=S[4]; t_prev=S[5];\n    F_ref=S[6]; x_ref_rig=S[7]; x_inicio=S[8]; u_prev=S[9]; modo_prev=S[10]; causa_act=S[11];\n} else {\n    x_ref=x; rig=rig_ini; F_pico=0; integ=0; sp_prev=med; t_prev=tr;\n    F_ref=F; x_ref_rig=x; x_inicio=x; u_prev=0; modo_prev=modo; causa_act=0;\n}\n\ndt_real = tr - t_prev;   /* periodo medido con el reloj del PC: solo diagnostico */\n\n/* estado del ensayo y reloj: se conservan aunque el resto del estado se reinicie */\nstp=0; f0p=0; tsp=0; inip=0; t=0;\nif (sizeOfDim(S,0)>=17) { stp=S[12]; f0p=S[13]; tsp=S[14]; inip=S[15]; t=S[16]; }\nt = t + dt;\nif (ini>0.5 && inip<0.5) t = dt;   /* el reloj del ensayo empieza con INICIAR */\n\nx_ref_ini = x_ref;   /* x_ref al empezar el paso (la proteccion de fuerza lo restituye) */\nprot = 0;\nst = stp;  f0 = f0p;  ts = tsp;\n\n/* ---------------------------------------------------------------------------\n   2. MAGNITUDES DERIVADAS Y LIMITES\n   --------------------------------------------------------------------------- */\n\n/* paro efectivo: boton PARO del panel o seta de emergencia pulsada */\nen_paro = 0;\nif (paro>0.5 || seta<0.5) en_paro = 1;\n\n/* fuerza estimada por las presiones [kN] y corte por presiones (hoy desactivado) */\nF_pres = cFpA*pa - cFpB*pb;\nlim_pres = 0;\nif (prot_pres_on>0.5 && (pa>=pa_max || F_pres>=F_corte)) lim_pres = 1;\n\n/* velocidad de aproximacion [mm/min] y limite de fuerza fuera de ensayo [kN] */\nv_aprox = vjog;\nif (v_aprox<=0) v_aprox = 25;\nv_aprox = min(50,v_aprox);\n\nF_lib = abs(Flib);\nif (F_lib<=0) F_lib = 4;\nF_lib = max(0.2,min(50,F_lib));\n\n/* ---------------------------------------------------------------------------\n   3. INICIO DEL ENSAYO\n   El ensayo arranca en el flanco de subida de INICIAR (ini = 1, inip = 0).\n   --------------------------------------------------------------------------- */\n\n/* reinicio sin salto al iniciar o al cambiar el tipo de control: la referencia se\n   iguala a la posicion y el integrador SE CONSERVA (guarda el null aprendido), asi\n   el comando sigue donde estaba. Ponerlo a cero mandaba 0 V durante 0.1-0.4 s */\nif ((ini>0.5 && inip<0.5) || modo!=modo_prev) {\n    x_ref = x;\n    sp_prev = med;\n}\n\n/* ---------------------------------------------------------------------------\n   4. GENERADOR DE CONSIGNA sp (maquina de estados)\n   --------------------------------------------------------------------------- */\nif (ini<0.5) {\n    /* FUERA DE ENSAYO: avance a v_aprox, retorno a v_retorno. Lento solo si se\n       avanza con compresion (F > frac_freno*F_lib); el retorno nunca se frena.\n       En fuerza, la consigna spm se limita a +-F_lib (o +-F_corte si sinprot). */\n    st = ST_REPOSO;\n    causa_act = CAU_NINGUNA;\n    if (modo>0.5) {\n        if (sinprot>0.5) {\n            dif = max(-F_corte,min(F_corte,spm)) - sp_prev;\n        } else {\n            dif = max(-F_lib,min(F_lib,spm)) - sp_prev;\n        }\n        vel_sp = v_des;\n    } else {\n        dif = spm - sp_prev;\n        vel_sp = v_aprox;\n        if (dif<0) vel_sp = v_retorno;\n        if (sinprot<0.5 && dif>0 && F>frac_freno*F_lib) vel_sp = min(v_aprox,v_lenta);\n    }\n    /* la consigna sigue a spm con pendiente limitada a vel_sp [unidad/min] */\n    sp = sp_prev + max(-vel_sp*dt/60,min(vel_sp*dt/60,dif));\n} else {\n    /* EN ENSAYO */\n    if (inip<0.5) {\n        /* primer paso del ensayo: arranca la carga desde la medicion actual */\n        st = ST_CARGA;\n        f0 = med;\n        ts = t;\n        F_pico = 0;\n        F_ref = F;\n        x_ref_rig = x;\n        x_inicio = x;\n        causa_act = CAU_NINGUNA;\n    }\n    dif = lim - f0;\n    if (st==ST_CARGA) {\n        /* carga: rampa hacia lim */\n        sp = f0 + sign(dif)*abs(rate)*(t-ts)/60;\n        if (dif*(sp-lim)>=0) { sp=lim; st=ST_MANTIENE; ts=t; }\n    } else if (st==ST_MANTIENE) {\n        /* mantener lim durante tc segundos */\n        sp = lim;\n        if (t-ts>=tc) { st=ST_DESCARGA; ts=t; }\n    } else if (st==ST_DESCARGA) {\n        /* descarga: a v_retorno [mm/min] en desplazamiento, a v_des [kN/min] en fuerza */\n        vel_sp = v_des;\n        if (modo<0.5) vel_sp = v_retorno;\n        sp = lim - sign(dif)*vel_sp*(t-ts)/60;\n        if (dif*(f0-sp)>=0) { sp=f0; st=ST_RETORNO; ts=t; }\n    } else {\n        /* retorno/fin (4) o FALLA (5): consigna en el valor inicial */\n        sp = f0;\n    }\n}\n\n/* ---------------------------------------------------------------------------\n   5. RIGIDEZ ESTIMADA rig = dF/dx\n   En linea en todo momento salvo retorno y falla (reposo, aproximacion, carga,\n   mantenimiento y descarga, en ambos modos): asi el lazo de fuerza usa la\n   rigidez real.\n   --------------------------------------------------------------------------- */\ndF_min = dF_min_rig;\nif (ini>0.5) dF_min = max(dF_min_rig,dF_min_rig*abs(lim-f0));\nif (st<=ST_DESCARGA && abs(F-F_ref)>dF_min && abs(x-x_ref_rig)>dx_min_rig) {\n    rig_nueva = (F-F_ref)/(x-x_ref_rig);\n    if (rig_nueva>rig_min) rig = rig + alfa_rig*(rig_nueva-rig);\n    F_ref = F;\n    x_ref_rig = x;\n}\nif (abs(x-x_ref_rig)>dx_sin_contacto) { F_ref=F; x_ref_rig=x; }   /* sin contacto: reinicia la referencia */\nrig = max(rig_min,min(rig_max,rig));\n\n\n/* ---------------------------------------------------------------------------\n   6. LAZO EXTERNO: consigna de posicion x_ref\n   --------------------------------------------------------------------------- */\nif (modo>0.5) {\n    /* control de fuerza */\n    if (st==ST_RETORNO) {\n        /* retorno a la posicion inicial x_inicio a v_retorno */\n        x_ref = x_ref + sign(x_inicio-x_ref)*min(abs(x_inicio-x_ref),v_retorno*dt/60);\n    } else if (st!=ST_FALLA) {\n        /* avance de x_ref en este paso: prealimentacion de la rampa + correccion\n           normalizada por rigidez, limitado a v_aprox (evita embalarse sin contacto) */\n        x_ref = x_ref + max(-v_aprox*dt/60,min(v_aprox*dt/60,(sp-sp_prev)/rig + Kf*(sp-F)/rig*dt));\n    }\n} else {\n    /* control de desplazamiento */\n    if (st!=ST_FALLA) x_ref = sp;\n}\n\n\n/* ---------------------------------------------------------------------------\n   7. PROTECCION DE FUERZA FUERA DE ENSAYO\n   Con compresion F > F_lib no deja avanzar; retroceder (alejarse) siempre esta\n   permitido.\n   --------------------------------------------------------------------------- */\nif (st==ST_REPOSO && sinprot<0.5) {\n    if (F>F_lib) { x_ref=min(x_ref,x_ref_ini); integ=min(integ,0); prot=1; }\n    if (prot>0.5 && modo<0.5) sp = x_ref;\n}\n\n\n/* ---------------------------------------------------------------------------\n   8. DETECCION DE FALLA, LIMITES Y PARO DE EMERGENCIA\n   --------------------------------------------------------------------------- */\nif (st>=ST_CARGA && st<=ST_DESCARGA) {\n    F_pico = max(F_pico,F);\n    if (modo>0.5 && st<=ST_MANTIENE && F_pico>frac_pico_min*abs(lim) && F<(1-frac_caida)*F_pico) {\n        st=ST_FALLA; causa_act=CAU_CAIDA; x_ref=x;           /* caida de carga */\n    } else if (modo>0.5 && F>frac_sobre*abs(lim)) {\n        st=ST_FALLA; causa_act=CAU_SOBRECARGA; x_ref=x;      /* sobrecarga */\n    } else if (x>xlim+margen_xlim) {\n        st=ST_FALLA; causa_act=CAU_LIM_POS; x_ref=x;         /* limite de posicion */\n    }\n}\n/* limite del sistema: en ensayo se declara FALLA */\nif (st>=ST_CARGA && st<=ST_RETORNO && abs(F)>=F_corte) { st=ST_FALLA; causa_act=CAU_FCORTE;  x_ref=x; }\nif (st>=ST_CARGA && st<=ST_RETORNO && lim_pres>0.5)    { st=ST_FALLA; causa_act=CAU_PRESION; x_ref=x; }\n/* bomba detenida durante el ensayo: FALLA (si la paro la seta o el PARO, manda esa causa) */\nif (st>=ST_CARGA && st<=ST_RETORNO && uph<0.5)         { st=ST_FALLA; causa_act=CAU_BOMBA;   x_ref=x; }\nif (en_paro>0.5 && ini>0.5)  { st=ST_FALLA; causa_act=CAU_PARO; }\nif (st==ST_FALLA) sp = med;\nif (modo>0.5) sp = max(-F_corte,min(F_corte,sp));   /* consigna de fuerza nunca sobre el corte */\n\n\n/* ---------------------------------------------------------------------------\n   9. LAZO INTERNO DE POSICION (PI con anti-windup) Y SEGURIDADES DE SALIDA\n   --------------------------------------------------------------------------- */\nx_ref = max(x-x_win,min(x+x_win,x_ref));\nerr = x_ref - x;\nu = Kx*(err+integ/Tix);\n/* integra solo si no satura y si de verdad esta controlando (ni paro ni bomba detenida) */\nif (abs(u)<u_max && en_paro<0.5 && uph>0.5) integ = integ + err*dt;\nu = max(-u_max,min(u_max,u));\nu = max(u_prev-du_max*dt,min(u_prev+du_max*dt,u));           /* limite de variacion (V/s) */\n\n/* LIMITE DEL SISTEMA: desde F_corte no se permite empujar mas, en cualquier estado y modo.\n   \"No empujar\" es u <= u_seguro: con 0 V el vastago seguiria extendiendose */\nif (F>=F_corte)  { u=min(u,u_seguro); integ=min(integ,0); x_ref=min(x_ref,x); prot=1; }\nif (F<=-F_corte) { u=max(u,0); integ=max(integ,0); x_ref=max(x_ref,x); prot=1; }\n/* corte por presiones (solo si prot_pres_on = 1) */\nif (lim_pres>0.5) { u=min(u,u_seguro); integ=min(integ,0); x_ref=min(x_ref,x); prot=1; }\n/* PARO o BOMBA DETENIDA: comando seguro y seguimiento, con el integrador congelado,\n   para que no haya salto al soltar el paro ni al arrancar la bomba (sin esto, con\n   la bomba parada el PI se iria a +-10 V y la valvula estaria abierta del todo en\n   el arranque) */\nif (en_paro>0.5 || uph<0.5) { u=u_seguro; x_ref=x; sp=med; }\n\n\n/* ---------------------------------------------------------------------------\n   10. INDICADORES PARA LA INTERFAZ\n   --------------------------------------------------------------------------- */\nprog = 0;\ntrest = 0;\nif (st==ST_MANTIENE) {\n    if (tc>0) prog = 100*min(1,(t-ts)/tc);\n    trest = max(0,tc-(t-ts));\n}\nif (st==ST_DESCARGA || st==ST_RETORNO) prog = 100;\nfalla = 0;\nif (st==ST_FALLA) falla = 1;\ncausa = causa_act;\nif (uph<0.5 && st!=ST_FALLA) causa = CAU_BOMBA;   /* aviso sin falla: por que no hay movimiento */\nif (en_paro>0.5) { causa=CAU_PARO; falla=1; }     /* alarma de PARO tambien fuera de ensayo */\n\n\n/* ---------------------------------------------------------------------------\n   11. ESTADO PARA EL SIGUIENTE PASO Y ESTADO PARA LA INTERFAZ Y EL REGISTRO\n   --------------------------------------------------------------------------- */\nsp_prev = sp;\nu_prev = u;\nt_prev = tr;      /* reloj del PC del paso (para dt_real) */\nmodo_prev = modo;\n\nSo[0]=x_ref;  So[1]=rig;       So[2]=F_pico;  So[3]=integ;     So[4]=sp_prev; So[5]=t_prev;\nSo[6]=F_ref;  So[7]=x_ref_rig; So[8]=x_inicio; So[9]=u_prev;   So[10]=modo_prev; So[11]=causa_act;\nSo[12]=st;    So[13]=f0;       So[14]=ts;      So[15]=ini;      So[16]=t;\n\nE[0]=t;    E[1]=st;   E[2]=sp;   E[3]=F;   E[4]=x;   E[5]=x_ref;\nE[6]=u;    E[7]=rig;  E[8]=dt;   E[9]=falla; E[10]=causa; E[11]=prot;\nE[12]=pa;  E[13]=pb;  E[14]=F_pres;\nE[15]=seta;   E[16]=uph;    E[17]=0;      E[18]=0;     E[19]=0;   E[20]=0;\nif (sizeOfDim(G,0)>=7) { E[17]=G[2]; E[18]=G[3]; E[19]=G[4]; E[20]=G[5]; }\nE[21]=F_pico; E[22]=prog;   E[23]=trest;  E[24]=act;   E[25]=aviso;\nE[26]=dt_real; E[27]=modo;\n\n\n/* ---------------------------------------------------------------------------\n   12. PROTECCION ANTE DATOS INVALIDOS\n   Medida invalida (ok = 0 o NaN en posicion o fuerza) o comandos incompletos:\n   salida u_seguro, FALLA en ensayo y reinicio del estado (So[1]=0 hace que el\n   proximo paso lo descarte).\n   --------------------------------------------------------------------------- */\nif (!(x==x) || !(F==F) || ok<0.5 || par_ok<0.5) {\n    u = u_seguro;\n    falla = 1;\n    So[1] = 0;\n    if (st>=ST_CARGA && st<=ST_RETORNO) st = ST_FALLA;\n    So[12] = st;\n    E[1] = st;\n    E[6] = u;\n    E[9] = 1;\n}"("M"=w276, "G"=w267, "C"=w240, "S"=w274, "tr"=w273) -> ("u"=w269:dbl, "So"=w275:dbl[], "E"=w252:dbl[])
    n108 = feedback-in #2(w275) -> ()
    n109 = Index Array(array=w252, index=1) -> (element=w251:dbl)
    n110 = call-poly <vilib>:"DAQmx Write.vi"("task/channels in"=w268, "data"=w269, "error in"=w253) -> ("task out"=w263:refnum<k21>, "error out"=w243:errorcluster)  [unwired: 10 in, 1 out]
    n111 = Greater?(x=w251, y=0.5) -> (0:w239:bool)
    n112 = call <extravilib>:"Write.vi"("element"=w252) -> ("channel"=w257:T3)  [unwired: 1 out]
    n113 = case shown="True" w239 {
      tunnel: w252 -> [_ w287]
      tunnel: [_ w283] -> w242
      frame False {
      }
      frame True {
        n114 = Array Subset(array=w287, index=0, length=15) -> (w284:dbl[])
        n115 = call <extravilib>:"Write.vi"("element"=w284) -> ("channel"=w283:T4)  [unwired: 8 in, 2 out]
      }
    }
    n116 = Unbundle By Name(w243) -> ("status"=w245:bool)
    n117 = Or(x=w246, y=w245) -> (x .or. y?=w244:bool)
  }
  n118 = call <vilib>:"DAQmx Stop Task.vi"("task/channels in"=w22) -> ("task out"=w24:refnum<k21>, "error out"=w14:errorcluster)  [unwired: 13 in]
  n119 = call <vilib>:"DAQmx Stop Task.vi"("task/channels in"=w21, "error in"=w13) -> ("task out"=w23:refnum<k21>, "error out"=w12:errorcluster)  [unwired: 12 in]
  n120 = call-poly <vilib>:"DAQmx Write.vi"("task/channels in"=w32, "data"=-0.5) -> ("task out"=w26:refnum<k21>, "error out"=w9:errorcluster)  [unwired: 11 in, 1 out]
  n121 = call-poly <vilib>:"DAQmx Write.vi"("task/channels in"=w31, "data"=bool[] [FALSE, FALSE, FALSE, FALSE, FALSE, TRUE, FALSE, FALSE]) -> ("task out"=w29:refnum<k21>, "error out"=w11:errorcluster)  [unwired: 11 in, 1 out]
  n122 = call <vilib>:"DAQmx Clear Task.vi"("task in"=w24, "error in"=w14) -> ("error out"=w6:errorcluster)  [unwired: 13 in]
  n123 = call <vilib>:"DAQmx Clear Task.vi"("task in"=w23, "error in"=w12) -> ("error out"=w5:errorcluster)  [unwired: 13 in]
  n124 = call <vilib>:"DAQmx Stop Task.vi"("task/channels in"=w26, "error in"=w9) -> ("task out"=w27:refnum<k21>, "error out"=w8:errorcluster)  [unwired: 12 in]
  n125 = call <vilib>:"DAQmx Stop Task.vi"("task/channels in"=w29, "error in"=w11) -> ("task out"=w28:refnum<k21>, "error out"=w10:errorcluster)  [unwired: 12 in]
  n126 = call <vilib>:"DAQmx Clear Task.vi"("task in"=w27, "error in"=w8) -> ("error out"=w3:errorcluster)  [unwired: 13 in]
  n127 = call <vilib>:"DAQmx Clear Task.vi"("task in"=w28, "error in"=w10) -> ("error out"=w4:errorcluster)  [unwired: 13 in]
  n128 = Merge Errors(w6, w5, w4, w3) -> (w7:errorcluster)
  n129 = call <vilib>:"Simple Error Handler.vi"("error in (no error)"=w7) -> ()  [unwired: 4 in, 5 out]
  n130 = while {
    shift-right: [w362] -> _
    shift-left: dbl[] [] -> [w364]
    shift-right: [w361] -> _
    shift-left: dbl[] [] -> [w363]
    tunnel: w20 -> [w327]
    tunnel: [w295] -> w1
    i -> [w329]
    stop <- "Stop" stop-if-true
    n131 = call <extravilib>:"Read.vi"("channel"=w327) -> ("element"=w326:dbl[])  [unwired: 1 in, 1 out]
    n132 = Index Array(array=w326) -> (element #1=→"Tiempo (s)":dbl, element #2=w291:dbl, element #3=w320:dbl, element #4=w299:dbl, element #5=w300:dbl, element #6=→"Consigna posicion interna (mm)":dbl, element #8=→"Rigidez estimada (kN/mm)":dbl, element #10=w315:dbl, element #11=→"Causa de la falla":dbl, element #12=w312:dbl, element #13=→"Presión A (bar)":dbl, element #14=→"Presión B (bar)":dbl, element #17=w308:dbl, element #19=w307:dbl, element #20=w304:dbl, element #21=w301:dbl, element #22=→"Carga maxima (kN)":dbl, element #23=→"Progreso mantenimiento":dbl, element #24=→"Tiempo restante carga (s)":dbl, element #25=→"Parametros avanzados":dbl, element #27=w293:dbl)  [unwired: 28 in, 7 out]
    "Fuerza actual (KN)" <- w299
    "Posicion actual (mm)" <- w300
    "Vertical Progress Bar" <- w300
    "Estado del ensayo" <- w291
    n133 = expression code="1000*x"(w293) -> (→"time/iteration (ms)":dbl)
    n134 = Not Equal To 0?(x=w315) -> (x != 0?=→"Falla":bool)
    n135 = Not Equal To 0?(x=w312) -> (x != 0?=→"Proteccion de fuerza activa":bool)
    n136 = Not Equal To 0?(x=w308) -> (x != 0?=→"Estado de motor":bool)
    n137 = Not Equal To 0?(x=w307) -> (x != 0?=→"Nivel tanque":bool)
    n138 = Equal To 0?(x=w304) -> (x = 0?=→"Estado de  filtro":bool)
    n139 = Not Equal To 0?(x=w301) -> (x != 0?=→"Sobrecorriente":bool)
    n140 = Equal To 0?(x=w301) -> (x = 0?=→"UPH energizada":bool)
    n141 = Greater?(x=w291, y=0.5) -> (0:w289:bool)
    n142 = call <vilib>:"Boolean Crossing PtByPt.vi"("input"=w289) -> ("crossing"=w290:bool)  [unwired: 2 in]
    n143 = global write "GlobalesPrensa.vi" "Ensayando"(w289) -> ()
    n144 = case shown="True" w290 {
      frame False {
      }
      frame True {
        n145 = property on="Tenacidad en vigas" class="Ring (strict)"() -> ("RingText.Text"=w370:string)  [unwired: 2 in, 2 out]
        n146 = global write "GlobalesPrensa.vi" "InfoEnsayo"(w370) -> ()
      }
    }
    n147 = local read "Tipo control"() -> (w297:u16)
    n148 = case shown="1" w297 {
      tunnel: [w374 w378] -> w296
      frame 0, Default {
        n149 = local read "Fuerza actual (KN)"() -> (w373:dbl)
        n150 = local read "Posicion actual (mm)"() -> (w374:dbl)
        n151 = property on="Fuerza deseada (kN)" class="DigNum (strict)"("DisabledEnum"=T5."Disabled" ("Disabled")) -> ()  [unwired: 2 in, 2 out]
        n152 = property on="Posicion deseada (mm)" class="Slide (strict)"("DisabledEnum"=T5."Enabled" ("Disabled")) -> ()  [unwired: 2 in, 2 out]
        n153 = local write "Fuerza deseada (kN)"(w373) -> ()
      }
      frame 1 {
        n154 = local read "Posicion actual (mm)"() -> (w377:dbl)
        n155 = local read "Fuerza actual (KN)"() -> (w378:dbl)
        n156 = local write "Posicion deseada (mm)"(w377) -> ()
        n157 = property on="Fuerza deseada (kN)" class="DigNum (strict)"("DisabledEnum"=T5."Enabled" ("Disabled")) -> ()  [unwired: 2 in, 2 out]
        n158 = property on="Posicion deseada (mm)" class="Slide (strict)"("DisabledEnum"=T5."Disabled" ("Disabled")) -> ()  [unwired: 2 in, 2 out]
      }
    }
    n159 = In Range and Coerce(upper limit=4.5, x=w291, lower limit=0.5) -> (In Range?=w354:bool)  [unwired: 1 out]
    n160 = Not Equal To 0?(x=w297) -> (x != 0?=w358:bool)
    n161 = Equal To 0?(x=w297) -> (x = 0?=w359:bool)
    n162 = Insert Into Array(array=w364, new element=w300) -> (w362:dbl[])  [unwired: 1 in]
    n163 = Insert Into Array(array=w363, new element=w299) -> (w361:dbl[])  [unwired: 1 in]
    n164 = case shown="1" "Tipo ensayos" {
      tunnel: [w381 w391] -> w357
      frame 0, Default {
        n165 = property on="Flexotracción en losas" class="Ring (strict)"("Visible"=TRUE) -> ()  [unwired: 2 in, 2 out]
        n166 = property on="Velocidad norma (mm/min)" class="DigNum (strict)"("Visible"=TRUE) -> ()  [unwired: 2 in, 2 out]
        n167 = case shown="0, Default" "Flexotracción en losas" {
          tunnel: [1.5 4.0 1.0 1.0] -> w381
          frame 0, Default {
          }
          frame 3 {
          }
          frame 2 {
          }
          frame 1 {
          }
        }
        "Velocidad norma (mm/min)" <- w381
        n168 = property on="Tenacidad en vigas" class="Ring (strict)"("Visible"=FALSE) -> ()  [unwired: 2 in, 2 out]
        n169 = property on="Velocidad norma (mm/min)  2" class="Str"("Visible"=FALSE) -> ()  [unwired: 2 in, 2 out]
      }
      frame 1 {
        n170 = property on="Tenacidad en vigas" class="Ring (strict)"("Visible"=TRUE) -> ()  [unwired: 2 in, 2 out]
        n171 = property on="Velocidad norma (mm/min)  2" class="Str"("Visible"=TRUE) -> ()  [unwired: 2 in, 2 out]
        n172 = case shown="2" "Tenacidad en vigas" {
          tunnel: ["0.05 - 0.1" "0.06 - 0.12" "0.1" "0.5 ± 0.05" "0.25"] -> w392
          frame 0, Default {
          }
          frame 1 {
          }
          frame 3 {
          }
          frame 4 {
          }
          frame 2 {
          }
        }
        "Velocidad norma (mm/min)  2" <- w392
        n173 = property on="Flexotracción en losas" class="Ring (strict)"("Visible"=FALSE) -> ()  [unwired: 2 in, 2 out]
        n174 = property on="Velocidad norma (mm/min)" class="DigNum (strict)"("Visible"=FALSE) -> ()  [unwired: 2 in, 2 out]
        n175 = Fract/Exp String To Number(string=w392) -> (number=w391:dbl)  [unwired: 3 in, 1 out]
      }
    }
    n176 = Not(x=w354) -> (.not. x?=w353:bool)
    n177 = property on="Rampa (mm/min)" class="DigNum (strict)"("Visible"=w359) -> ()  [unwired: 2 in, 2 out]
    n178 = property on="Rampa (kN/min)" class="DigNum (strict)"("Visible"=w358) -> ()  [unwired: 2 in, 2 out]
    n179 = property on="Limite fuerza (kN)" class="DigNum (strict)"("Visible"=w358) -> ()  [unwired: 2 in, 2 out]
    n180 = And(x="Aplicar velocidad de norma", y=w353) -> (x .and. y?=w351:bool)
    n181 = Bundle(w362, w361) -> (→"fuerza desplazamiento":cluster{dbl[], dbl[]})  [unwired: 1 in]
    n182 = Merge Signals(w320, w296) -> (→"control signals":dynamicdata)
    n183 = local read "Iniciar ensayo"() -> (w298:bool)
    n184 = Select(t=T5."Disabled" ("Disabled"), s=w298, f=T5."Enabled" ("Disabled")) -> (s? t:f=w365:T5)
    n185 = case shown="True" w351 {
      tunnel: w357 -> [_ w371]
      frame False {
      }
      frame True {
        n186 = local write "Rampa (mm/min)"(w371) -> ()
        n187 = local write "Tipo control"(enum16{"Desplazamiento", "Fuerza"}."Desplazamiento" ("Tipo control")) -> ()
      }
    }
    n188 = property on="Fuerza deseada (kN)" class="DigNum (strict)"("DisabledEnum"=w365) -> ()  [unwired: 2 in, 2 out]
    n189 = property on="Posicion deseada (mm)" class="Slide (strict)"("DisabledEnum"=w365) -> ()  [unwired: 2 in, 2 out]
    n190 = property on="Tiempo carga (s)" class="DigNum (strict)"("DisabledEnum"=w365) -> ()  [unwired: 2 in, 2 out]
    n191 = property on="Limite posicion (mm)" class="DigNum (strict)"("DisabledEnum"=w365) -> ()  [unwired: 2 in, 2 out]
    n192 = property on="Limite fuerza (kN)" class="DigNum (strict)"("DisabledEnum"=w365) -> ()  [unwired: 2 in, 2 out]
    n193 = property on="Rampa (kN/min)" class="DigNum (strict)"("DisabledEnum"=w365) -> ()  [unwired: 2 in, 2 out]
    n194 = Wait (ms)(milliseconds to wait=u32 100) -> ()  [unwired: 1 out]
    n195 = global write "GlobalesPrensa.vi" "Salir"("Stop") -> ()
    n196 = Build Array("Iniciar ensayo", "PARO DE EMERGENCIA", "Encender", "Apagar", "Stop", "Sin proteccion de carga") -> (w343:bool[])
    n197 = Boolean To (0,1)(Boolean=w343) -> (0, 1=w344:i16[])
    n198 = Build Array (concatenate)("Tipo control", w344, "Posicion deseada (mm)", "Fuerza deseada (kN)", "Limite posicion (mm)", "Limite fuerza (kN)", "Rampa (mm/min)", "Rampa (kN/min)", "Tiempo carga (s)", "Vel. aproximacion (mm/min)", "Fmax fuera de ensayo (kN)", "Codigo acceso", "Kx lazo posicion (V/mm)", "Ti lazo posicion (s)", "Kf lazo fuerza (1/s)", w329) -> (w328:dbl[])
    n199 = call <extravilib>:"Write.vi"("element"=w328) -> ("channel"=w295:T6)  [unwired: 1 out]
  }
  n200 = while {
    tunnel: w2 -> [w407]
    stop <- w403 stop-if-true
    n201 = call <extravilib>:"Read.vi"("timeout in ms (-1)"=100, "channel"=w407) -> ("element"=w404:dbl[], "element valid?"=w405:bool)  [unwired: 5 in, 3 out]
    n202 = case shown="True" w405 {
      tunnel: w404 -> [_ w408]
      frame False {
      }
      frame True {
        n203 = global read "GlobalesPrensa.vi" "ArchivoControl"() -> (w411:path)
        n204 = call-poly <vilib>:"Write Delimited Spreadsheet.vi"("file path (dialog if empty)"=w411, "format (%.3f)"="%.5f", "1D data"=w408, "append to file? (new file:F)"=TRUE) -> ()  [unwired: 10 in, 2 out]
      }
    }
    n205 = global read "GlobalesPrensa.vi" "Salir"() -> (w403:bool)
  }
